vi "VM - Test Context.vi"(8 "error in":errorcluster, 11 "VC Handle":T1=-1) -> (0 "error out":errorcluster, 1 "err code":T2 items=["No error", "Invalid variable type", "Variable not found", "Variable already exists", "Invalid context handle", "Input error", "Invalid data format", "No history attached", "History already attached", "Invalid history parameters", "Wrong variable name", "Wrong alias name", "Non-unique alias", "Alias not found", "No alias associated", "Alias already associated", "Wrong context name", "Non-unique context name", "Context name not found", "Invalid parameter", "Generic error", "Memory Full", "Unrecognized LV error", "Unknown error code"], 3 "dup VC Handle":T1=-1)   [LabVIEW 2021]
doc: "<b>*** DEPRECATED ***</b>\n\nThe VI tests a handle of variables context.\n\n<VC Handle> control has to contain a handle to be tested. VI returns an error if the handle doesn't correspond to opened context.\n\n::: CalcExpress Toolkit :::\nCopyright (c) 2000-2026 Konstantin Shifershteyn. All rights reserved."
uses:
  cetypes.llb/VarMan Variable Context Handle.ctl
  cetypes.llb/VarMan Error Code.ctl
  cersrc/celveng32.dll
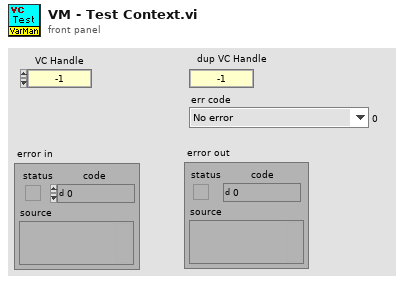
[diagram p1: front panel]
types:
  T1 = typedef "VarMan Variable Context Handle.ctl" = i32
  T2 = typedef "VarMan Error Code.ctl" = u16
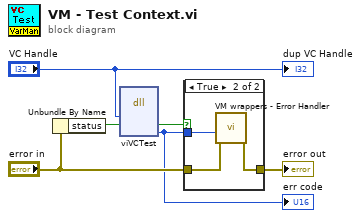
[diagram p0: block diagram]
diagram:
  n1 = Unbundle By Name("error in") -> ("status"=w4:bool)
  n2 = dll-call lib="C:/LV Projects/CalcExpress 40 LV2021/vi.lib/addons/CalcExpress/cersrc/celveng*.dll" fn="viVCTest"("vch"="VC Handle", "errf"=w4) -> ("errf"=w2:bool, "err code"=w3:T2)  [unwired: 6 in, 2 out]
  "err code" <- w3
  n3 = case shown="True" w2 {
    tunnel: [w7 w10] -> w6
    tunnel: "error in" -> [w7 w9]
    tunnel: w3 -> [_ w8]
    frame False {
    }
    frame True {
      n4 = call "VM wrappers - Error Handler.vi"("error before"=w9, "VarMan error"=w8) -> ("error out"=w10:errorcluster)  [unwired: 8 in, 1 out]
    }
  }
  "error out" <- w6
  "dup VC Handle" <- "VC Handle"
